vi "Show.vi"(8 "error in (no error)":errorcluster, 10 "ToastSource in":refnum<class "ToastSource.lvclass">, 11 "ToastService in":refnum<class "ToastService.lvclass">) -> (0 "error out":errorcluster, 3 "ToastService out":refnum<class "ToastService.lvclass">)   [LabVIEW 2026, in "ToastNotification.lvlib" / "ToastService.lvclass"]
doc: "Display a borrowed ToastSource by dynamically invoking its Show implementation. Skipped on incoming error; return the same service and propagate errors. Register the service activation handler before display if replies are required. Does not initialize, retain or close the source. Keep its existing class value for caller-owned cleanup after its last use."
uses:
  ToastService.lvclass
  ToastSource/ToastSource.lvclass
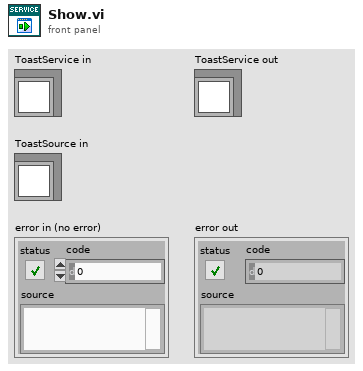
[diagram p1: front panel]
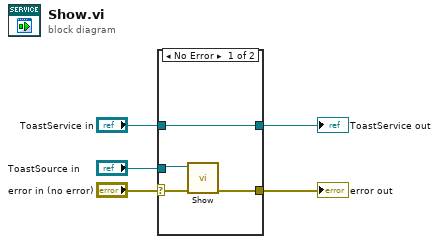
[diagram p0: block diagram]
diagram:
  n1 = case shown="No Error" "error in (no error)" {
    selector: "error in (no error)" -> [w8 w11]
    tunnel: "ToastService in" -> [w9 w10]
    tunnel: [w9 w10] -> w3
    tunnel: [w6 w11] -> w2
    tunnel: "ToastSource in" -> [w7 _]
    frame No Error {
      n2 = call-dynamic "Show.vi"("error in (no error)"=w8, "ToastSource in"=w7) -> ("error out"=w6:errorcluster)  [unwired: 8 in, 1 out]
    }
    frame Error {
    }
  }
  "ToastService out" <- w3
  "error out" <- w2
